vi "SubSystem Wizard New.vi"() -> ()   [LabVIEW 2027]
panel:
  in  "Description":string
  in  "Color":u32(colorbox)
  in  "Operations":i32(listbox)
  in  "Boolean 4":bool
  in  "Boolean 3":bool
  in  "Boolean 2":bool
  in  "Boolean":bool
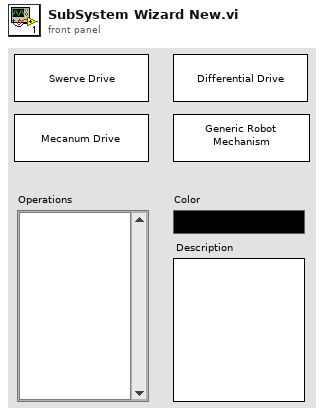
[diagram p1: front panel]
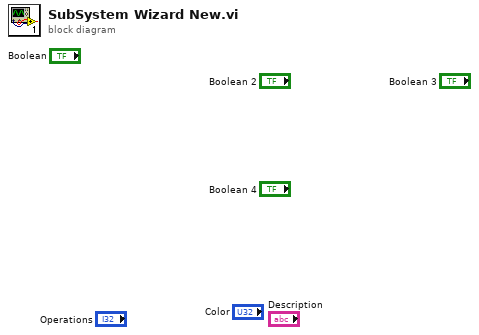
[diagram p0: block diagram]
diagram:
